vi "Prepare Config Reload.vi"(8 "error in (no error)":errorcluster, 9 "Reload Options":T1, 11 "Volatus Core in":refnum<class "Volatus Core.lvclass">) -> (0 "error out":errorcluster, 3 "Volatus Core out":refnum<class "Volatus Core.lvclass">)   [LabVIEW 2020, in "Volatus.lvlib" / "Volatus Core.lvclass"]
uses:
  Volatus Core.lvclass
  C:/dev/lv20CE/relink/lv-volatus/Volatus/Module/Module.lvclass
  Reload Options.ctl
  Config Updater/Config Updater.lvclass
  Reload State.ctl
  Volatus Core.lvclass/Volatus Core.ctl
  Module/Module.lvclass/Module.ctl
  Module/Module.lvclass
  Volatus.lvlib
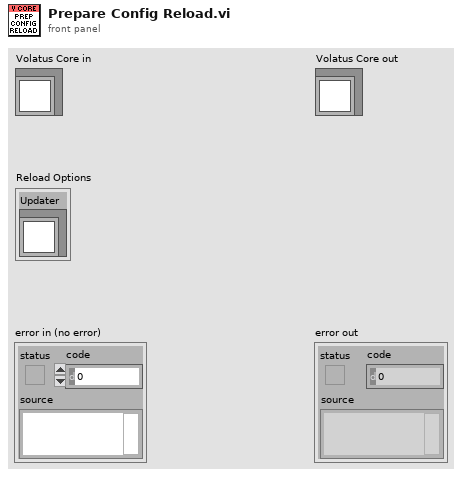
[diagram p1: front panel]
types:
  T1 = typedef "Volatus.lvlib/Reload Options.ctl" = cluster{"Updater":refnum<class "Config Updater.lvclass">}
  T2 = typedef "Volatus.lvlib/Volatus Core.lvclass/Reload State.ctl" = enum16{"None", "Stop Modules", "Close Vecto", "Reload", "Restart"}
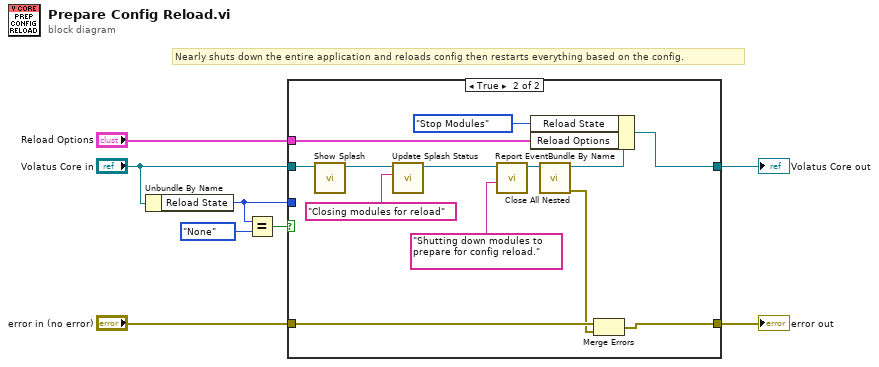
[diagram p0: block diagram]
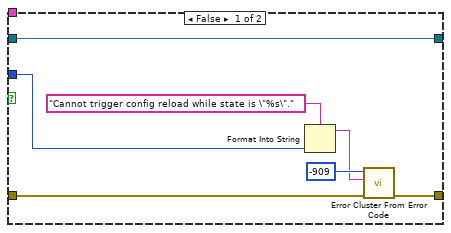
[diagram p2: hidden frame]
diagram:
  # "Nearly shuts down the entire application and reloads config then restarts everything based on the config."
  n1 = Unbundle By Name("Volatus Core in") -> ("Reload State"=w2:T2)
  n2 = Equal?(x=w2, y=Reload_State."None") -> (x = y?=w6:bool)
  n3 = case shown="True" w6 {
    tunnel: "Volatus Core in" -> [w9 w28]
    tunnel: [w9 w25] -> w5
    tunnel: "error in (no error)" -> [w15 w27]
    tunnel: [w14 w26] -> w3
    tunnel: w2 -> [w11 _]
    tunnel: "Reload Options" -> [_ w23]
    frame False {
      n4 = Format Into String(format string="Cannot trigger config reload while state is \"%s\".", w11) -> (resulting string=w10:string)  [unwired: 2 in, 1 out]
      n5 = call <vilib>:"Error Cluster From Error Code.vi"("error in (no error)"=w15, "error message (\"\")"=w10, "error code (0)"=-909) -> ("error out"=w14:errorcluster)  [unwired: 6 in]
    }
    frame True {
      n6 = call "Show Splash.vi"("Volatus Core in"=w28) -> ("Volatus Core out"=w18:refnum<class "Volatus Core.lvclass">)  [unwired: 9 in, 1 out]
      n7 = call "Update Splash Status.vi"("Status"="Closing modules for reload", "Volatus Core in"=w18) -> ("Volatus Core out"=w17:refnum<class "Volatus Core.lvclass">)  [unwired: 8 in, 1 out]
      n8 = call "Report Event.vi"("Message"="Shutting down modules to prepare for config reload.", "Module in"=w17) -> ("Module out"=w20:refnum<class "Volatus Core.lvclass">)  [unwired: 8 in, 1 out]
      n9 = call "Close All Nested.vi"("Module in"=w20) -> ("error out"=w21:errorcluster, "Module out"=w22:refnum<class "Volatus Core.lvclass">)  [unwired: 9 in]
      n10 = Bundle By Name(cluster=w22, "Reload State"=Reload_State."Stop Modules", "Reload Options"=w23) -> (w25:refnum<class "Volatus Core.lvclass">)
      n11 = Merge Errors(w27, w21) -> (w26:errorcluster)
    }
  }
  "error out" <- w3
  "Volatus Core out" <- w5
